vi "P-733 XY Stage Engine.vi"(0 "Notifier Name":string, 11 "Axis Names":string[](array[string])) -> ()   [LabVIEW 2016]
uses:
  Stages Controls/Stage Notifier Element.ctl
  Stages Controls/Stage Actions.ctl
  Stages Controls/Stage Status.ctl
  PI GCS2 DLL/PI_GCS2_DLL_x64.dll
panel:
  in  "Velocity":dbl=5.0
  out "current v":dbl[](array[numeric])
  out "target pos":dbl[](array[numeric])
  out "Success":u32
  in  "Right":bool
  in  "Left":bool
  in  "Y Position (µm)":dbl format="%#.3g"
  in  "Down":bool
  in  "Up":bool
  in  "X Position (µm)":dbl format="%#.3g"
  in  "Step Size (µm)":dbl=0.1
  in  "QUIT":bool
  in  "Abort":bool
  out "P-733 Found":bool
  out "Number Connected":i32
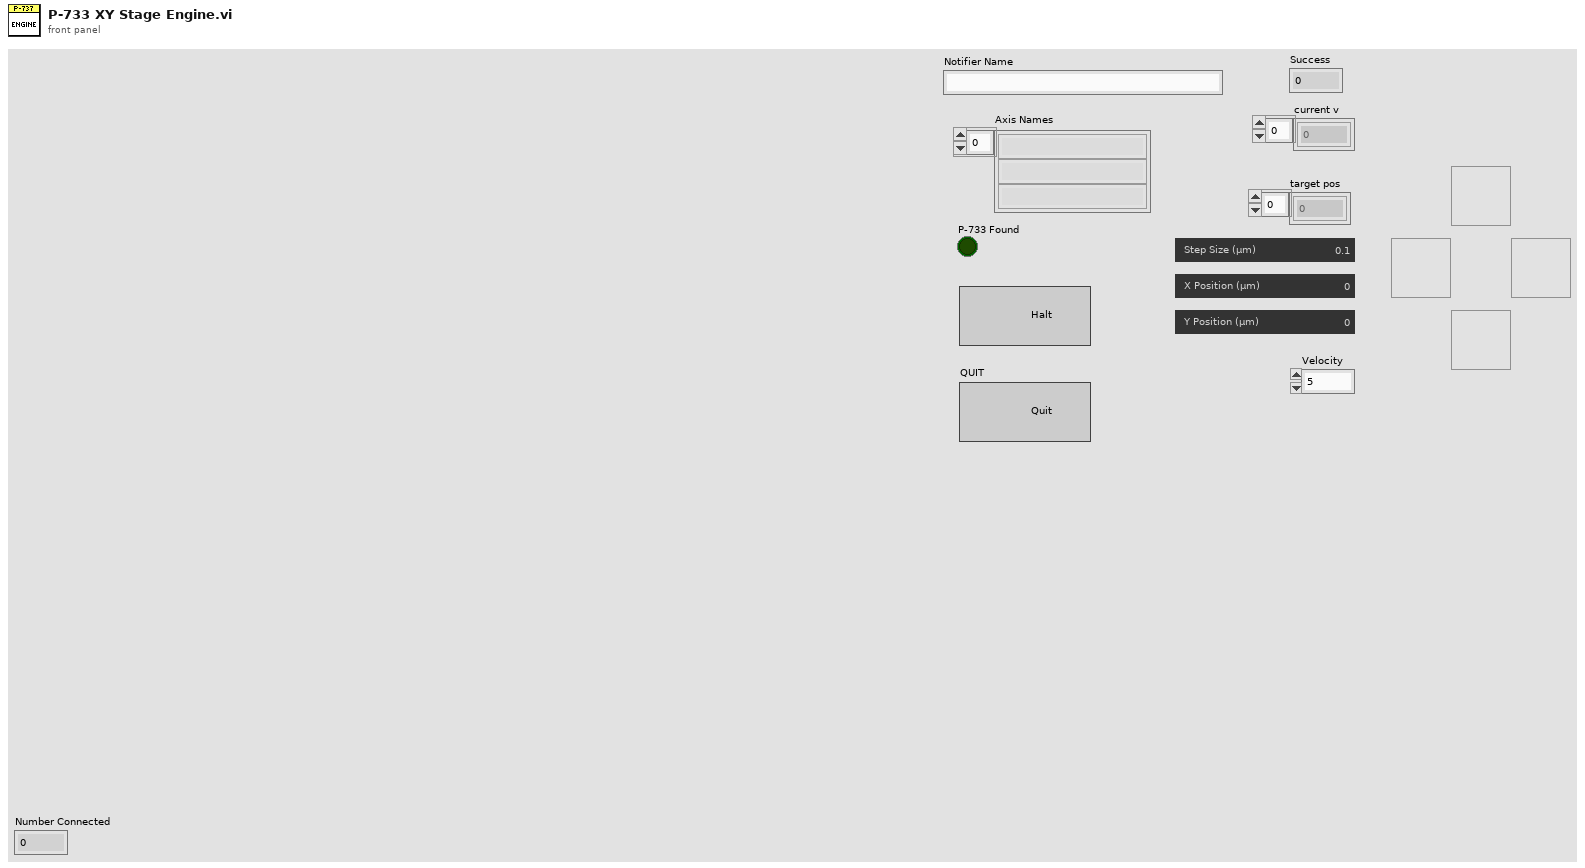
[diagram p1: front panel]
types:
  T1 = typedef "Stage Notifier Element.ctl" = cluster{"Action":T2, "Axis":bool[], "Setpoint":dbl[], "Velocity":dbl, "Cmd Recvd?":bool, "Position":dbl[], "Status":T3, "Misc":variant}
  T2 = typedef "Stage Actions.ctl" = enum16{"Get Position", "MVR", "MOVE", "HALT", "ONTARGET", "ERROR", "REFERENCE", "INIT", "VELOCITY", "STATUS", "EXIT", "HOME", "ZEROPOS", "NANOPOS", "ANALOG", "QUIT"}
  T3 = typedef "Stage Status.ctl" = enum16{"Error", "Abort", "Busy", "On Target"}
  T4 = enum32{"Invalid", "Standard", "Closed", "Hidden", "Minimized", "Maximized"}
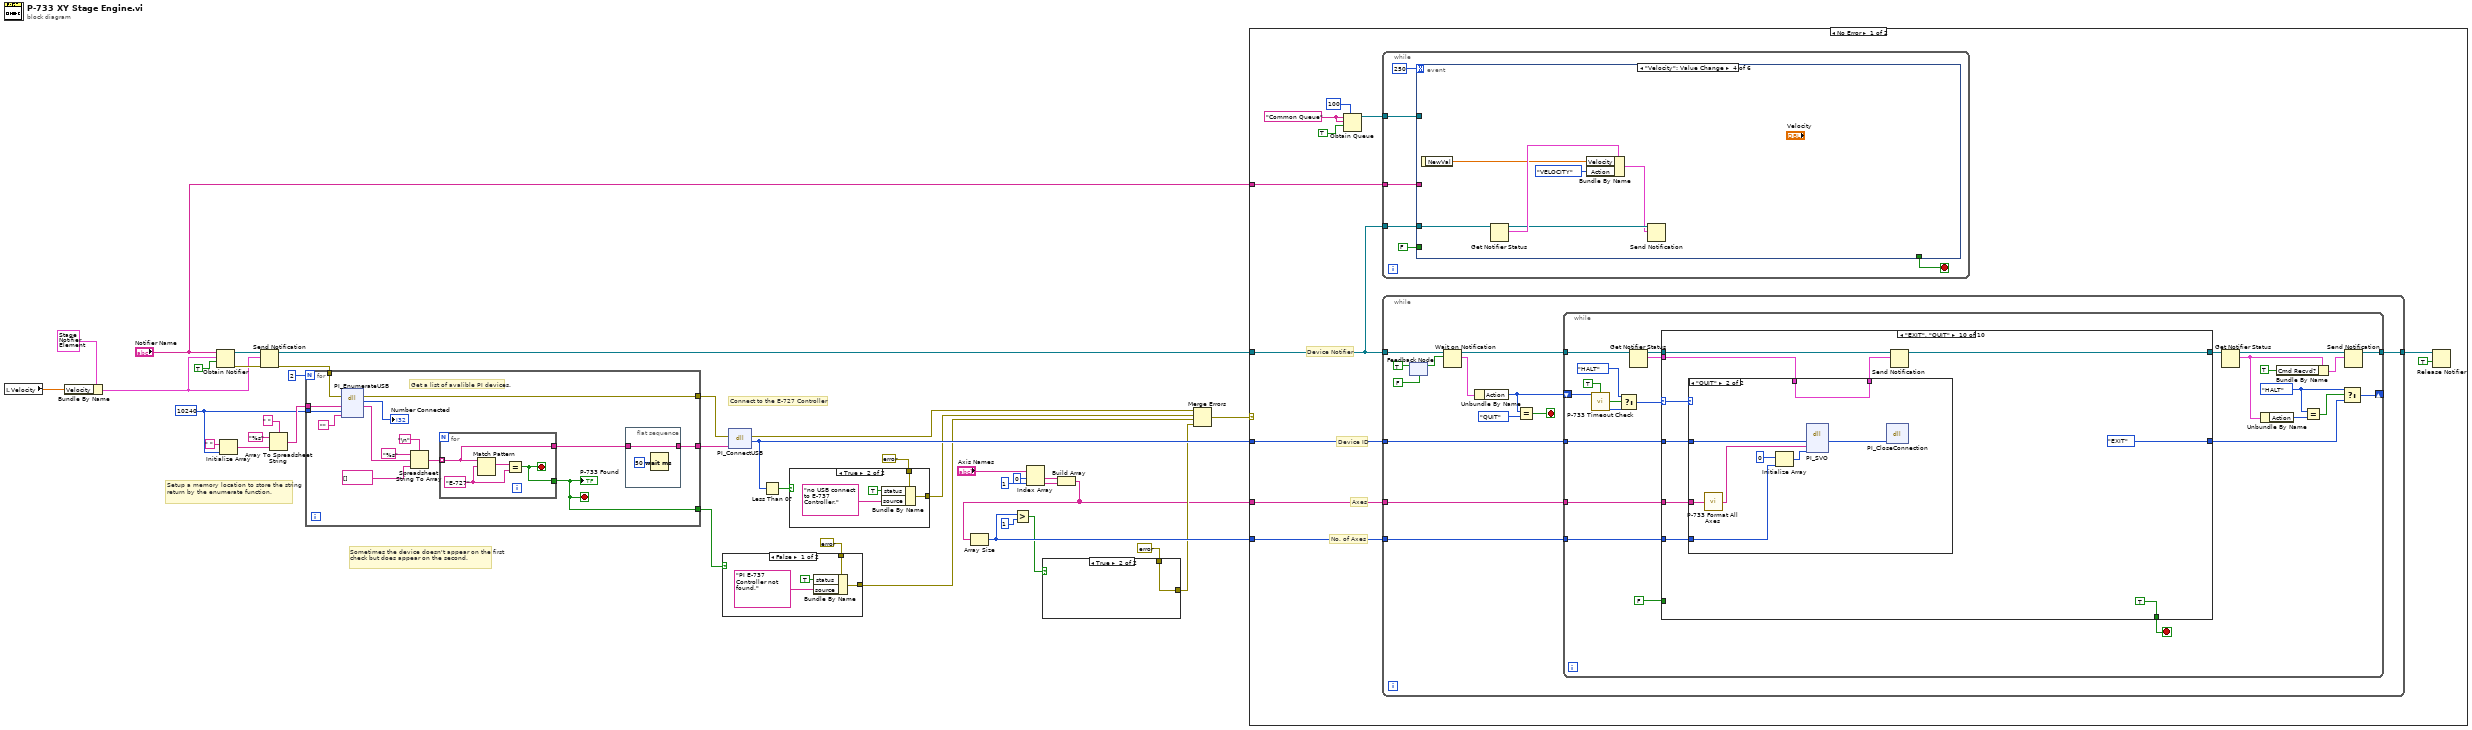
[diagram p0: block diagram]
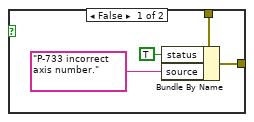
[diagram p2: hidden frame]
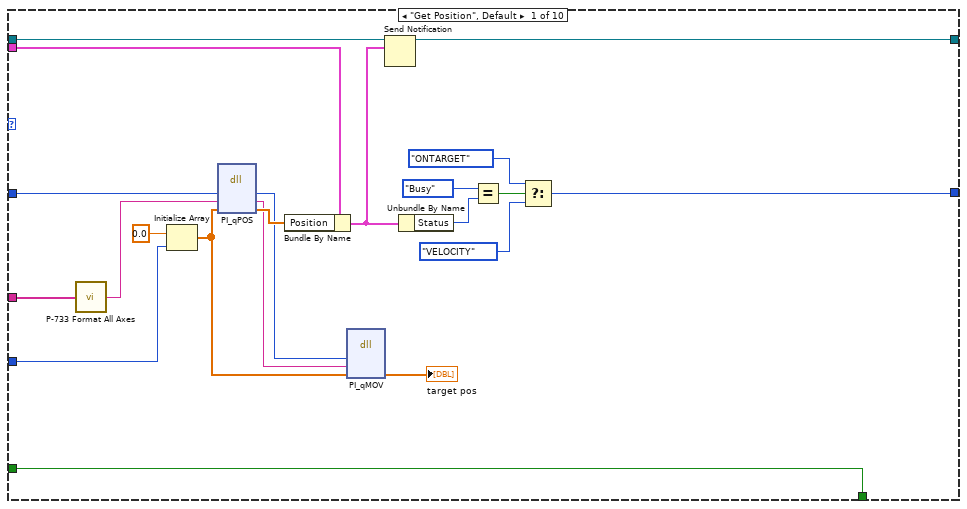
[diagram p5: hidden frame]
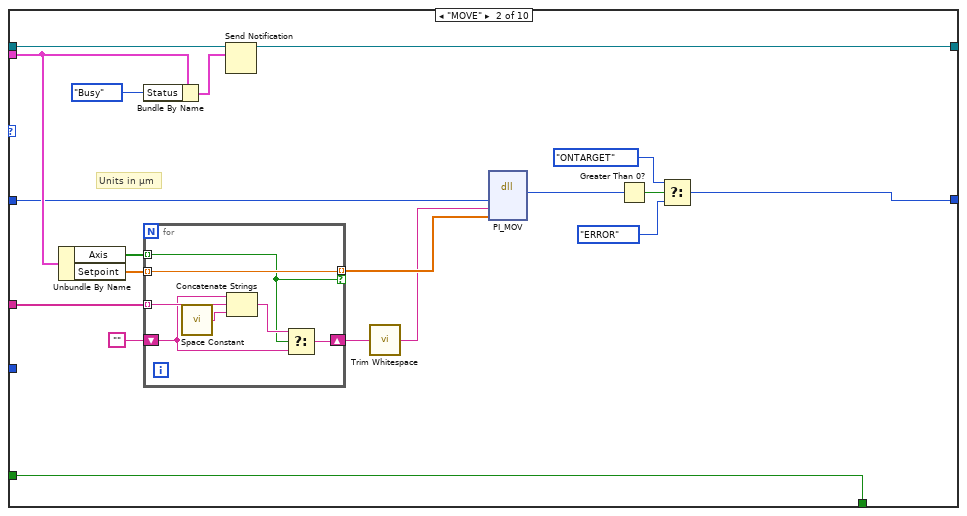
[diagram p6: hidden frame]
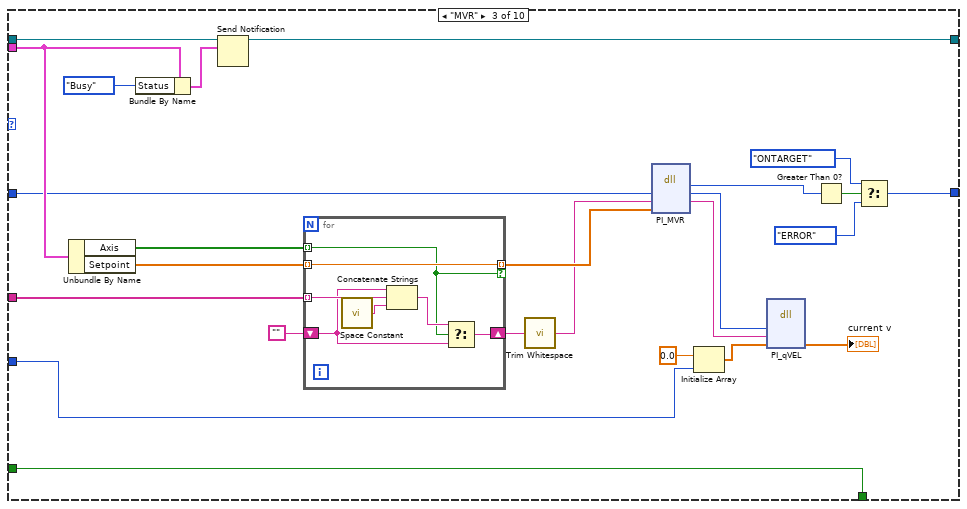
[diagram p7: hidden frame]
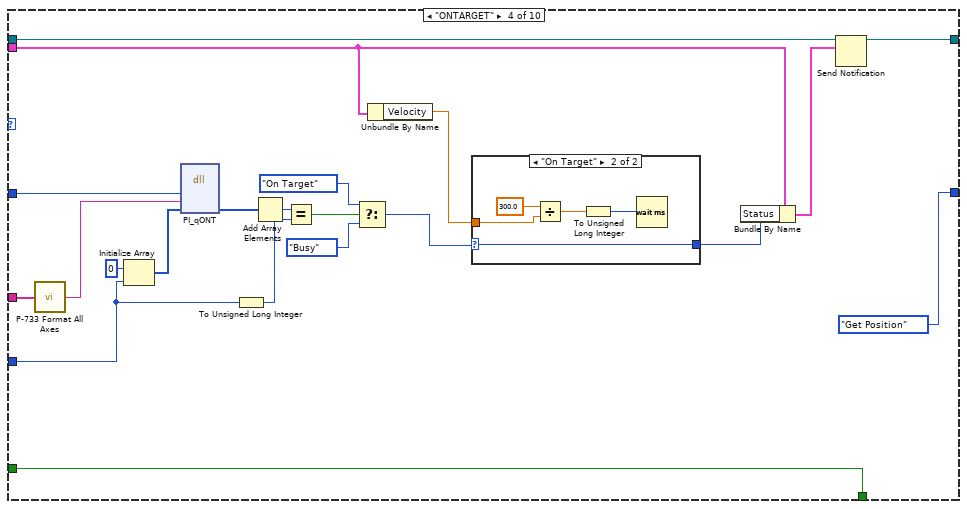
[diagram p8: hidden frame]
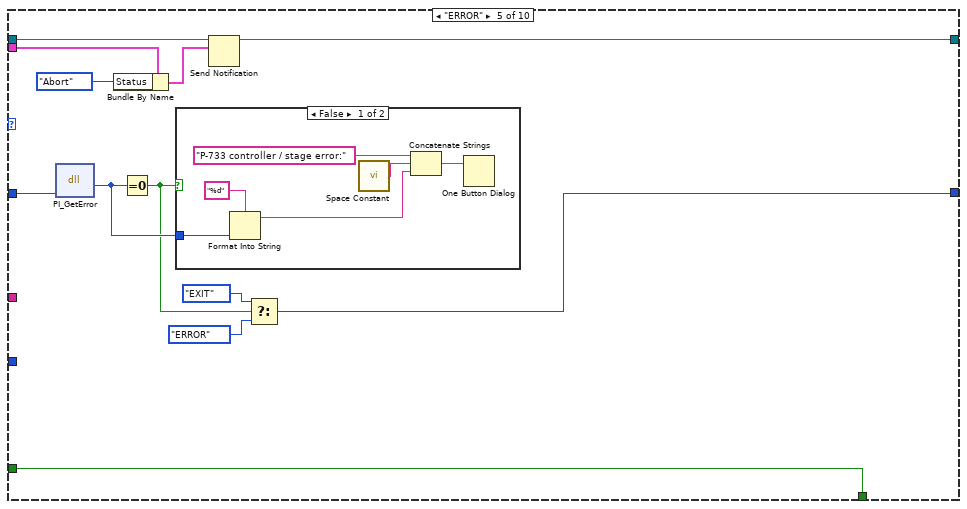
[diagram p10: hidden frame]
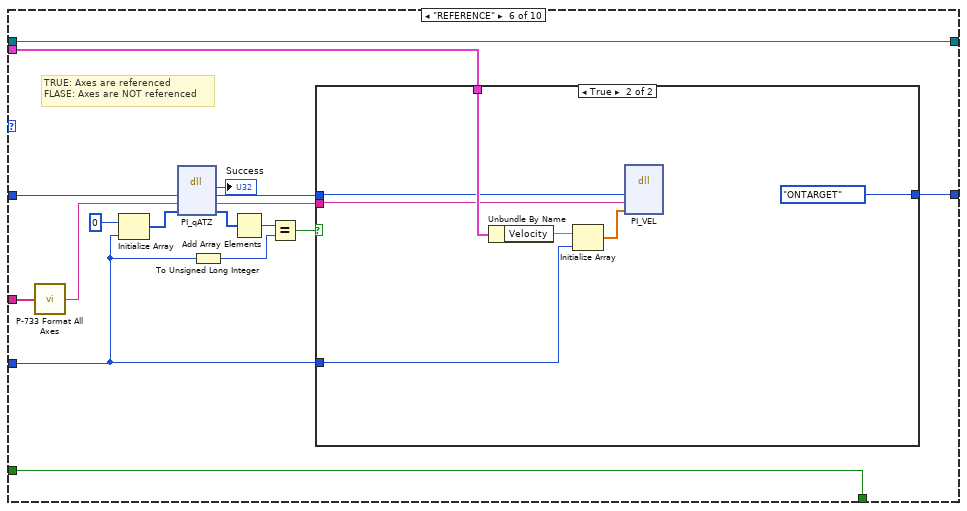
[diagram p12: hidden frame]
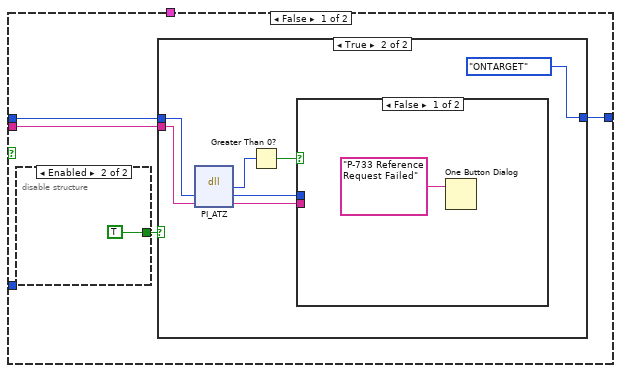
[diagram p13: hidden frame]
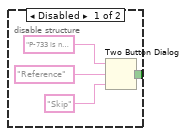
[diagram p14: hidden frame]
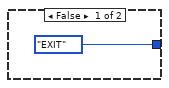
[diagram p15: hidden frame]
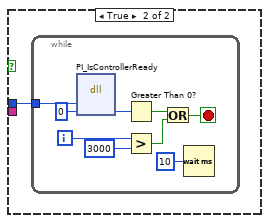
[diagram p16: hidden frame]
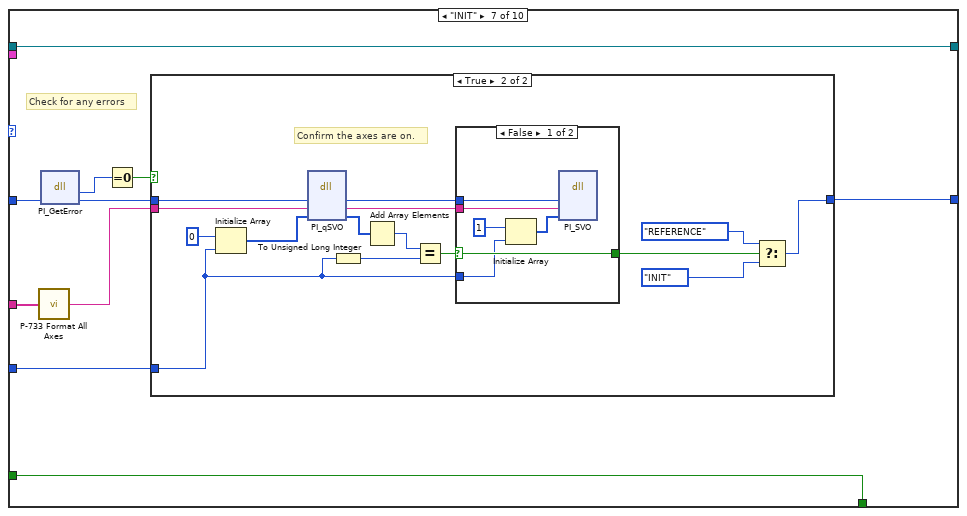
[diagram p17: hidden frame]
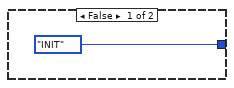
[diagram p18: hidden frame]
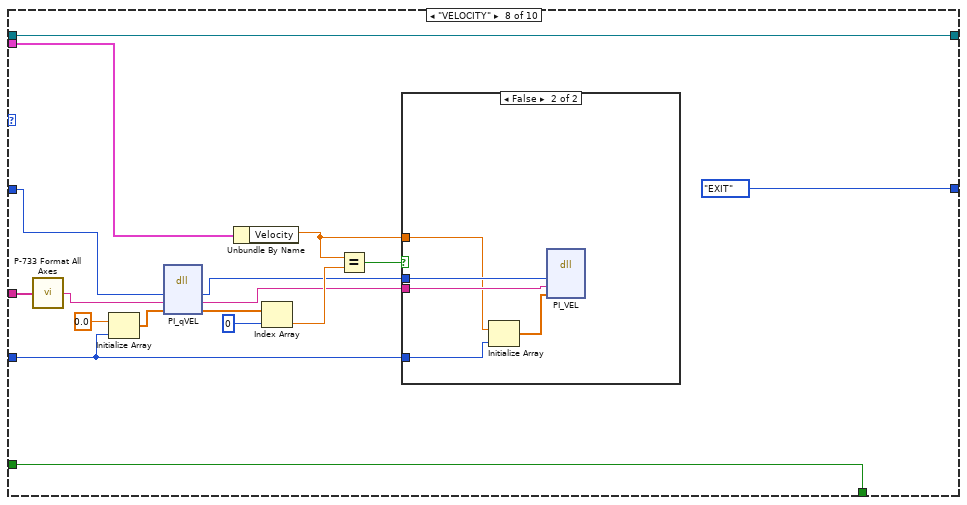
[diagram p20: hidden frame]
diagram:
  w33 = 10240 ("dimension size")
  # "Setup a memory location to store the string return by the enumerate function."
  # "Connect to the E-727 Controller"
  # "Sometimes the device doesn't appear on the first check but does appear on the second."
  n1 = local read "Velocity"() -> (w1:dbl)
  n2 = Bundle By Name(cluster=T1 {"Action"=enum."INIT", "Axis"=[], "Setpoint"=[], "Velocity"=5.0, "Cmd Recvd?"=FALSE, "Position"=[], "Status"=enum."Error", "Misc"=variant} ("Stage Status"), "Velocity"=w1) -> (w2:T1)
  n3 = Obtain Notifier(name (unnamed)="Notifier Name", notification data type=w2, create if not found? (T)=TRUE) -> (notifier out=w19:refnum<notifier>, error out=w18:errorcluster)  [unwired: 1 in, 1 out]
  n4 = Initialize Array(" ", w33) -> (w37:string[])
  n5 = Send Notification(notification=w2, notifier=w19, error in (no error)=w18) -> (notifier out=w16:refnum<notifier>, error out=w17:errorcluster)
  n6 = Array To Spreadsheet String(delimiter (Tab)=" ", array=w37, 3:"%s" ("format string")) -> (spreadsheet string=w34:string)
  n7 = for {
    N: 2 -> [_]
    tunnel: w34 -> [w47]
    tunnel: w33 -> [w46]
    tunnel: [w42] -> w31
    tunnel: [w41] -> w25
    tunnel: [w40] -> w30
    tunnel: w17 -> [w39]
    stop <- w41 stop-if-true
    # "Get a list of avalible PI devices."
    n8 = dll-call lib="C:/Users/Ries Lab/Documents/Microscope Control from Sheng Account/Microscope-Control/Device Library/Stages/PI/PI GCS2 DLL/PI_GCS2_DLL_x64.dll" fn="PI_EnumerateUSB"(error in=w39, "szBuffer"=w47, "iBufferSize"=w46, "szFilter"="") -> (error out=w40:errorcluster, "return type"=→"Number Connected":i32, "szBuffer"=w44:string)  [unwired: 4 in, 1 out]
    n9 = Spreadsheet String To Array(delimiter (Tab)="\n", format string="%s", spreadsheet string=w44, array type (2D Dbl)=string[] []) -> (array=w49:string[])
    n10 = for {
      tunnel: w49 -> [w56] mode=indexing
      tunnel: [w56] -> w43
      tunnel: [w55] -> w41
      stop <- w55 stop-if-true
      w57 = "E-727"
      n11 = Match Pattern(string=w56, regular expression=w57) -> (match substring=w58:string)  [unwired: 1 in, 3 out]
      n12 = Equal?(x=w58, y=w57) -> (x = y?=w55:bool)
    }
    "P-733 Found" <- w41
    n13 = flat-sequence {
      tunnel: w43 -> [w54]
      tunnel: [w54] -> w42
      frame #0 {
        n14 = Wait (ms)(milliseconds to wait=u32 50) -> ()  [unwired: 1 out]
      }
    }
  }
  n15 = case shown="False" w25 {
    tunnel: errorcluster {"status"=FALSE, "code"=0, "source"=""} ("error in (no error)") -> [w60 w63]
    tunnel: [w59 w63] -> w21
    frame False {
      n16 = Bundle By Name(cluster=w60, "status"=TRUE, "source"="PI E-737 Controller not found.") -> (w59:errorcluster)
    }
    frame True {
    }
  }
  n17 = dll-call lib="C:/Users/Ries Lab/Documents/Microscope Control from Sheng Account/Microscope-Control/Device Library/Stages/PI/PI GCS2 DLL/PI_GCS2_DLL_x64.dll" fn="PI_ConnectUSB"(error in=w30, "szDescription"=w31) -> (error out=w23:errorcluster, "Device ID"=w28:i32)  [unwired: 3 in, 1 out]
  n18 = Less Than 0?(x=w28) -> (x < 0?=w27:bool)
  n19 = case shown="True" w27 {
    tunnel: errorcluster {"status"=FALSE, "code"=0, "source"=""} ("error in (no error)") -> [w64 w68]
    tunnel: [w64 w65] -> w22
    frame False {
    }
    frame True {
      n20 = Bundle By Name(cluster=w68, "status"=TRUE, "source"="no USB connect to E-737 Controller.") -> (w65:errorcluster)
    }
  }
  n21 = Index Array(array="Axis Names", index #1=0 ("index"), index #2=1 ("index")) -> (element #1=w6:string, element #2=w5:string)
  n22 = Build Array(w6, w5) -> (w4:string[])
  n23 = Array Size(array=w4) -> (size(s)=w13:i32)
  n24 = Greater?(x=w13, y=1) -> (0:w11:bool)
  n25 = case shown="True" w11 {
    tunnel: errorcluster {"status"=FALSE, "code"=0, "source"=""} ("error in (no error)") -> [w70 w73]
    tunnel: [w69 w73] -> w10
    frame False {
      n26 = Bundle By Name(cluster=w70, "status"=TRUE, "source"="P-733 incorrect axis number.") -> (w69:errorcluster)
    }
    frame True {
    }
  }
  n27 = Merge Errors(w23, w22, w21, w10) -> (w20:errorcluster)
  n28 = case shown="No Error" w20 {
    selector: w20 -> [_ w484]
    tunnel: w16 -> [w78 w486]
    tunnel: "Notifier Name" -> [w79 _]
    tunnel: w28 -> [w77 w485]
    tunnel: w4 -> [w75 _]
    tunnel: w13 -> [w74 _]
    frame No Error {
      w83 = "Common Queue" ("Unique Notifier Name")
      # "Device Notifier"
      # "No. of Axes"
      # "Axes"
      # "Device ID"
      n29 = Obtain Queue(max queue size (-1, unlimited)=100, name (unnamed)=w83, element data type=w83, create if not found? (T)=TRUE) -> (queue out=w80:refnum<queue>)  [unwired: 1 in, 2 out]
      n30 = while {
        tunnel: w78 -> [w386]
        tunnel: w80 -> [w385]
        tunnel: w79 -> [w384]
        stop <- w387 stop-if-true
        n31 = event shown="[3] \"Velocity\": Value Change" {
          selector: _ -> [_ _ _ _ _ _]
          dyn-events: _ -> [_ _ _ _ _ _]
          timeout: 250 -> [_ _ _ _ _ _]
          tunnel: [w398 w407 w425 _ w453 w476] -> w387
          tunnel: w386 -> [w404 _ w418 w439 w445 w479]
          tunnel: w385 -> [w400 _ _ _ _ _]
          tunnel: w384 -> [w395 _ _ _ _ _]
          tunnel: FALSE -> [_ w407 w425 _ w453 w476]
          event Timeout {
            # "Notification with QUIT command"
            n32 = event-data() -> ()  [unwired: 1 in, 1 out]
            n33 = call "Common Device Queue Get Command.vi"("Common Queue"=w400, "Notifier Name"=w395) -> ("Command"=w401:string)  [unwired: 12 in, 1 out]
            n34 = control-ref of="This VI"() -> (w402:refnum<vi>)
            n35 = Get Notifier Status(notifier=w404) -> (notifier out=w396:refnum<notifier>, current notification=w394:T1, error out=w403:errorcluster)  [unwired: 1 in, 2 out]
            n36 = call "Common Device Queue Execute Command.vi"("Common Command"=w401, "VI Refnum"=w402) -> ("Quit?"=w397:bool)  [unwired: 12 in, 1 out]
            n37 = Unbundle By Name(w403) -> ("status"=w399:bool)
            n38 = case shown="True" w397 {
              tunnel: w396 -> [_ w406]
              frame False {
              }
              frame True {
                n39 = Send Notification(notification=T1 {"Action"=enum."QUIT", "Axis"=[], "Setpoint"=[], "Velocity"=5.0, "Cmd Recvd?"=FALSE, "Position"=[], "Status"=enum."Error", "Misc"=variant} ("Stage Status"), notifier=w406) -> ()  [unwired: 1 in, 2 out]
              }
            }
            n40 = Or(x=w397, y=w399) -> (x .or. y?=w398:bool)
            n41 = Unbundle By Name(w394) -> ("Position"=w393:dbl[])
            n42 = Index Array(array=w393, index #1=0 ("index"), index #2=1 ("index")) -> (element #1=w389:dbl, element #2=w390:dbl)
            n43 = local write "X Position (µm)"(w389) -> ()
            n44 = local write "Y Position (µm)"(w390) -> ()
          }
          event Application Instance Close? {
            n45 = event-data() -> ()  [unwired: 1 in, 5 out]
            n46 = control-ref of="This VI"() -> (w409:refnum<vi>)
            n47 = invoke class="VI" method="FP.Open"(reference=w409, "Activate"=TRUE ("Activate?"), "State"=T4."Standard") -> ()  [unwired: 2 in, 5 out]
            n48 = event-data("Discard?"=TRUE) -> ()  [unwired: 1 in, 1 out]
          }
          event "X Position (µm)", "Y Position (µm)": Value Change {
            n49 = event-data() -> ("CtlRef"=w424:refnum<vi>, "NewVal"=w422:dbl)  [unwired: 1 in]
            n50 = Build Array(w422, 0.0) -> (w420:dbl[])
            n51 = property class="DigNum (strict)"(reference=w424) -> ("Label.Text"=w423:string)  [unwired: 1 in, 2 out]
            n52 = case shown="\"Y Position (µm)\"" w423 {
              tunnel: w420 -> [_ w429 w433]
              tunnel: bool[] [TRUE, FALSE] -> [_ w428 w431]
              tunnel: [dbl[] [0.0, 0.0] w429 w432] -> w414
              tunnel: [bool[] [FALSE, FALSE] w428 w430] -> w413
              frame Default {
              }
              frame "X Position (µm)" {
              }
              frame "Y Position (µm)" {
                n53 = Reverse 1D Array(array=w433) -> (reversed array=w432:dbl[])
                n54 = Reverse 1D Array(array=w431) -> (reversed array=w430:bool[])
              }
            }
            n55 = Get Notifier Status(notifier=w418) -> (notifier out=w417:refnum<notifier>, current notification=w416:T1)  [unwired: 1 in, 3 out]
            n56 = Bundle By Name(cluster=w416, "Action"=Stage_Actions."MOVE", "Setpoint"=w414, "Axis"=w413) -> (w412:T1)
            n57 = Send Notification(notification=w412, notifier=w417) -> ()  [unwired: 1 in, 2 out]
          }
          event "Velocity": Value Change {
            n58 = event-data() -> ("NewVal"=w437:dbl)  [unwired: 1 in]
            n59 = Get Notifier Status(notifier=w439) -> (notifier out=w436:refnum<notifier>, current notification=w438:T1)  [unwired: 1 in, 3 out]
            n60 = Bundle By Name(cluster=w438, "Velocity"=w437, "Action"=Stage_Actions."VELOCITY") -> (w435:T1)
            n61 = Send Notification(notification=w435, notifier=w436) -> ()  [unwired: 1 in, 2 out]
          }
          event "Up", "Down", "Left", "Right": Value Change {
            n62 = event-data() -> ("CtlRef"=w448:refnum<vi>)  [unwired: 1 in]
            n63 = property class="Bool"(reference=w448) -> ("Label.Text"=w447:string)  [unwired: 1 in, 2 out]
            n64 = Build Array("Step Size (µm)", 0.0 ("element")) -> (w450:dbl[])
            n65 = case shown="\"Left\", \"Right\"" w447 {
              selector: w447 -> [_ w462 w468]
              tunnel: w450 -> [_ w459 w467]
              tunnel: bool[] [TRUE, FALSE] -> [_ w456 w465]
              tunnel: [dbl[] [0.0, 0.0] w458 w464] -> w442
              tunnel: [bool[] [FALSE, FALSE] w456 w463] -> w441
              frame Default {
              }
              frame "Down", "Up" {
                n66 = Negate(x=w459) -> (-x=w460:dbl[])
                n67 = Equal?(x=w462, y="Down") -> (x = y?=w457:bool)
                n68 = Select(t=w460, s=w457, f=w459) -> (s? t:f=w458:dbl[])
              }
              frame "Left", "Right" {
                n69 = Reverse 1D Array(array=w465) -> (reversed array=w463:bool[])
                n70 = Negate(x=w467) -> (-x=w470:dbl[])
                n71 = Equal?(x=w468, y="Left") -> (x = y?=w469:bool)
                n72 = Select(t=w470, s=w469, f=w467) -> (s? t:f=w466:dbl[])
                n73 = Reverse 1D Array(array=w466) -> (reversed array=w464:dbl[])
              }
            }
            n74 = Get Notifier Status(notifier=w445) -> (notifier out=w446:refnum<notifier>, current notification=w444:T1)  [unwired: 1 in, 3 out]
            n75 = Bundle By Name(cluster=w444, "Action"=Stage_Actions."MVR" ("Actions"), "Setpoint"=w442, "Axis"=w441) -> (w440:T1)
            n76 = Send Notification(notification=w440, notifier=w446) -> ()  [unwired: 1 in, 2 out]
          }
          event "QUIT", "Abort": Value Change {
            n77 = event-data() -> ("CtlRef"=w478:refnum<vi>)  [unwired: 1 in]
            n78 = property class="Bool"(reference=w478) -> ("Label.Text"=w477:string)  [unwired: 1 in, 2 out]
            n79 = case shown="\"QUIT\"" w477 {
              tunnel: [Stage_Actions."EXIT" ("Action") Stage_Actions."QUIT" ("Action") Stage_Actions."HALT" ("Action")] -> w475
              frame "Default", Default {
              }
              frame "QUIT" {
              }
              frame "Abort" {
              }
            }
            n80 = Get Notifier Status(notifier=w479) -> (notifier out=w473:refnum<notifier>, current notification=w472:T1)  [unwired: 1 in, 3 out]
            n81 = Bundle By Name(cluster=w472, "Action"=w475) -> (w474:T1)
            n82 = Send Notification(notification=w474, notifier=w473) -> ()  [unwired: 1 in, 2 out]
          }
        }
      }
      n83 = while {
        tunnel: w78 -> [w96]
        tunnel: w77 -> [w95]
        tunnel: [w93] -> w76
        tunnel: w75 -> [w91]
        tunnel: w74 -> [w90]
        stop <- w92 stop-if-true
        n84 = feedback #1(FALSE) -> (w86:bool)
        n85 = feedback-in #1(TRUE ("ignore previous (F)")) -> ()
        n86 = Wait on Notification(notifier=w96, ignore previous (F)=w86) -> (notifier out=w85:refnum<notifier>, notification=w94:T1)  [unwired: 2 in, 2 out]
        n87 = Unbundle By Name(w94) -> ("Action"=w89:T2)
        n88 = Equal?(x=w89, y=Stage_Actions."QUIT") -> (x = y?=w92:bool)
        n89 = while {
          tunnel: w95 -> [w120]
          tunnel: w85 -> [w117]
          shift-right: [w119] -> _
          shift-left: w89 -> [w113]
          tunnel: [w99] -> w93
          tunnel: w91 -> [w107]
          tunnel: w90 -> [w108]
          stop <- w121 stop-if-true
          w104 = Stage_Actions."HALT" ("t")
          n90 = call "P-733 Timeout Check.vi"("Action"=w113, "User Input?"=TRUE) -> ("Timeout?"=w112:bool, "Action (Dup)"=w111:T2)  [unwired: 12 in]
          n91 = Select(t=Stage_Actions."HALT" ("y"), s=w112, f=w111) -> (s? t:f=w110:T2)
          n92 = Get Notifier Status(notifier=w117) -> (notifier out=w116:refnum<notifier>, current notification=w115:T1)  [unwired: 1 in, 3 out]
          n93 = case shown="\"EXIT\", \"QUIT\"" w110 {
            selector: w110 -> [_ _ _ _ _ _ _ _ _ w371]
            tunnel: w116 -> [w132 w146 w181 w211 w233 w263 w302 w348 w361 w369]
            tunnel: FALSE -> [w142 w162 w194 w222 w240 w262 w306 w347 w354 _]
            tunnel: [w142 w162 w194 w222 w240 w262 w306 w347 w354 TRUE] -> w121
            tunnel: [w136 w158 w190 Stage_Actions."Get Position" ("y") w234 w258 w303 Stage_Actions."EXIT" ("y") Stage_Actions."ERROR" ("y") Stage_Actions."EXIT" ("y")] -> w118
            tunnel: w120 -> [w130 w155 w178 w207 w239 w261 w308 w337 w363 w372]
            tunnel: [w131 w144 w179 w210 w232 w263 w302 w348 w359 w367] -> w106
            tunnel: w115 -> [w135 w156 w188 w203 w231 w248 _ w346 w362 w370]
            tunnel: w108 -> [w124 _ w173 w218 _ w247 w299 w332 _ w364]
            tunnel: w107 -> [w133 w151 w185 w212 _ w251 w301 w344 w357 w365]
            frame "Get Position", Default {
              n94 = call "P-733 Format All Axes.vi"("All Axis Array"=w133) -> ("All Axes String"=w129:string)  [unwired: 14 in]
              n95 = Initialize Array(0.0 ("element"), w124) -> (w126:dbl[])
              n96 = dll-call lib="C:/Users/Ries Lab/Documents/Microscope Control from Sheng Account/Microscope-Control/Device Library/Stages/PI/PI GCS2 DLL/PI_GCS2_DLL_x64.dll" fn="PI_qPOS"("Device ID"=w130, "szAxes"=w129, "pdValueArray"=w126) -> ("Device ID"=w128:i32, "szAxes"=w127:string, "pdValueArray"=w134:dbl[])  [unwired: 4 in, 2 out]
              n97 = Bundle By Name(cluster=w135, "Position"=w134) -> (w123:T1)
              n98 = dll-call lib="C:/Users/Ries Lab/Documents/Microscope Control from Sheng Account/Microscope-Control/Device Library/Stages/PI/PI GCS2 DLL/PI_GCS2_DLL_x64.dll" fn="PI_qMOV"("ID"=w128, "szAxis"=w127, "pdValueArray"=w126) -> ("pdValueArray"=→"target pos":dbl[])  [unwired: 6 in, 2 out]
              n99 = Send Notification(notification=w123, notifier=w132) -> (notifier out=w131:refnum<notifier>)  [unwired: 1 in, 1 out]
              n100 = Unbundle By Name(w123) -> ("Status"=w141:T3)
              n101 = Equal?(x=Stage_Status."Busy", y=w141) -> (x = y?=w139:bool)
              n102 = Select(t=Stage_Actions."ONTARGET" ("y"), s=w139, f=Stage_Actions."VELOCITY" ("y")) -> (s? t:f=w136:T2)
            }
            frame "MOVE" {
              # "Units in µm"
              n103 = Unbundle By Name(w156) -> ("Axis"=w153:bool[], "Setpoint"=w152:dbl[])
              n104 = Bundle By Name(cluster=w156, "Status"=Stage_Status."Busy") -> (w145:T1)
              n105 = for {
                tunnel: w153 -> [w165] mode=indexing
                tunnel: w152 -> [w166] mode=indexing
                tunnel: w151 -> [w169] mode=indexing
                shift-right: [w164] -> w148
                shift-left: "" -> [w163]
                tunnel: [w166] -> w149 mode=indexing if=w165
                n106 = call <vilib>:"Space Constant.vi"() -> ("String"=w168:string)
                n107 = Concatenate Strings(w163, w169, w168) -> (w167:string)
                n108 = Select(t=w167, s=w165, f=w163) -> (s? t:f=w164:string)
              }
              n109 = Send Notification(notification=w145, notifier=w146) -> (notifier out=w144:refnum<notifier>)  [unwired: 1 in, 1 out]
              n110 = call <vilib>:"Trim Whitespace.vi"("string"=w148) -> ("trimmed string"=w147:string)  [unwired: 1 in]
              n111 = dll-call lib="C:/Users/Ries Lab/Documents/Microscope Control from Sheng Account/Microscope-Control/Device Library/Stages/PI/PI GCS2 DLL/PI_GCS2_DLL_x64.dll" fn="PI_MOV"("Device ID"=w155, "szAxes"=w147, "pdValueArray"=w149) -> ("Success"=w154:u32)  [unwired: 6 in, 2 out]
              n112 = Greater Than 0?(x=w154) -> (x > 0?=w161:bool)
              n113 = Select(t=Stage_Actions."ONTARGET" ("Action"), s=w161, f=Stage_Actions."ERROR" ("Action")) -> (s? t:f=w158:T2)
            }
            frame "MVR" {
              n114 = Unbundle By Name(w188) -> ("Axis"=w186:bool[], "Setpoint"=w170:dbl[])
              n115 = Bundle By Name(cluster=w188, "Status"=Stage_Status."Busy") -> (w180:T1)
              n116 = Send Notification(notification=w180, notifier=w181) -> (notifier out=w179:refnum<notifier>)  [unwired: 1 in, 1 out]
              n117 = for {
                tunnel: w186 -> [w197] mode=indexing
                tunnel: w170 -> [w198] mode=indexing
                tunnel: w185 -> [w201] mode=indexing
                shift-right: [w196] -> w182
                shift-left: "" -> [w195]
                tunnel: [w198] -> w183 mode=indexing if=w197
                n118 = call <vilib>:"Space Constant.vi"() -> ("String"=w200:string)
                n119 = Concatenate Strings(w195, w201, w200) -> (w199:string)
                n120 = Select(t=w199, s=w197, f=w195) -> (s? t:f=w196:string)
              }
              n121 = call <vilib>:"Trim Whitespace.vi"("string"=w182) -> ("trimmed string"=w177:string)  [unwired: 1 in]
              n122 = dll-call lib="C:/Users/Ries Lab/Documents/Microscope Control from Sheng Account/Microscope-Control/Device Library/Stages/PI/PI GCS2 DLL/PI_GCS2_DLL_x64.dll" fn="PI_MVR"("Device ID"=w178, "szAxes"=w177, "pdValueArray"=w183) -> ("Success"=w187:u32, "Device ID"=w176:i32, "szAxes"=w175:string)  [unwired: 4 in, 2 out]
              n123 = Initialize Array(0.0 ("element"), w173) -> (w172:dbl[])
              n124 = dll-call lib="C:/Users/Ries Lab/Documents/Microscope Control from Sheng Account/Microscope-Control/Device Library/Stages/PI/PI GCS2 DLL/PI_GCS2_DLL_x64.dll" fn="PI_qVEL"("Device ID"=w176, "szAxes"=w175, "pdValueArray"=w172) -> ("pdValueArray"=→"current v":dbl[])  [unwired: 6 in, 2 out]
              n125 = Greater Than 0?(x=w187) -> (x > 0?=w193:bool)
              n126 = Select(t=Stage_Actions."ONTARGET" ("Action"), s=w193, f=Stage_Actions."ERROR" ("Action")) -> (s? t:f=w190:T2)
            }
            frame "ONTARGET" {
              n127 = call "P-733 Format All Axes.vi"("All Axis Array"=w212) -> ("All Axes String"=w209:string)  [unwired: 14 in]
              n128 = Initialize Array(u32 0 ("element"), w218) -> (w208:u32[])
              n129 = dll-call lib="C:/Users/Ries Lab/Documents/Microscope Control from Sheng Account/Microscope-Control/Device Library/Stages/PI/PI GCS2 DLL/PI_GCS2_DLL_x64.dll" fn="PI_qONT"("Device ID"=w207, "szAxes"=w209, "pdValueArray"=w208) -> ("pdValueArray"=w220:u32[])  [unwired: 6 in, 2 out]
              n130 = To Unsigned Long Integer(number=w218) -> (unsigned 32bit integer=w217:u32)
              n131 = Add Array Elements(numeric array=w220) -> (sum=w219:u32)
              n132 = Equal?(x=w219, y=w217) -> (x = y?=w216:bool)
              n133 = Select(t=Stage_Status."On Target" ("Status"), s=w216, f=Stage_Status."Busy" ("Status")) -> (s? t:f=w206:T3)
              n134 = Unbundle By Name(w203) -> ("Velocity"=w202:dbl)
              n135 = case shown="\"On Target\"" w206 {
                selector: w206 -> [w223 w228]
                tunnel: [w223 w228] -> w204
                tunnel: w202 -> [_ w226]
                frame "Busy", Default {
                }
                frame "On Target" {
                  n136 = Divide(x=300.0, y=w226) -> (x/y=w225:dbl)
                  n137 = To Unsigned Long Integer(number=w225) -> (unsigned 32bit integer=w224:u32)
                  n138 = Wait (ms)(milliseconds to wait=w224) -> ()  [unwired: 1 out]
                }
              }
              n139 = Bundle By Name(cluster=w203, "Status"=w204) -> (w205:T1)
              n140 = Send Notification(notification=w205, notifier=w211) -> (notifier out=w210:refnum<notifier>)  [unwired: 1 in, 1 out]
            }
            frame "ERROR" {
              n141 = dll-call lib="C:/Users/Ries Lab/Documents/Microscope Control from Sheng Account/Microscope-Control/Device Library/Stages/PI/PI GCS2 DLL/PI_GCS2_DLL_x64.dll" fn="PI_GetError"("Device ID"=w239) -> ("Error Code"=w238:i32)  [unwired: 4 in, 2 out]
              n142 = Bundle By Name(cluster=w231, "Status"=Stage_Status."Abort") -> (w230:T1)
              n143 = Equal To 0?(x=w238) -> (x = 0?=w237:bool)
              n144 = case shown="False" w237 {
                tunnel: w238 -> [w244 _]
                frame False {
                  n145 = Format Into String(format string="%d", w244) -> (resulting string=w242:string)  [unwired: 2 in, 1 out]
                  n146 = call <vilib>:"Space Constant.vi"() -> ("String"=w245:string)
                  n147 = Concatenate Strings("P-733 controller / stage error:", w245, w242) -> (w241:string)
                  n148 = One Button Dialog(message=w241) -> ()  [unwired: 1 in, 1 out]
                }
                frame True {
                }
              }
              n149 = Send Notification(notification=w230, notifier=w233) -> (notifier out=w232:refnum<notifier>)  [unwired: 1 in, 1 out]
              n150 = Select(t=Stage_Actions."EXIT", s=w237, f=Stage_Actions."ERROR" ("Action")) -> (s? t:f=w234:T2)
            }
            frame "REFERENCE" {
              # "TRUE: Axes are referenced\nFLASE: Axes are NOT referenced"
              n151 = call "P-733 Format All Axes.vi"("All Axis Array"=w251) -> ("All Axes String"=w250:string)  [unwired: 14 in]
              n152 = Initialize Array(u32 0 ("element"), w247) -> (w259:u32[])
              n153 = dll-call lib="C:/Users/Ries Lab/Documents/Microscope Control from Sheng Account/Microscope-Control/Device Library/Stages/PI/PI GCS2 DLL/PI_GCS2_DLL_x64.dll" fn="PI_qATZ"("Device ID"=w261, "szAxes"=w250, "pdValueArray"=w259) -> ("Success"=→"Success":u32, "Device ID"=w256:i32, "szAxes"=w257:string, "pdValueArray"=w255:u32[])  [unwired: 3 in, 2 out]
              n154 = To Unsigned Long Integer(number=w247) -> (unsigned 32bit integer=w253:u32)
              n155 = Add Array Elements(numeric array=w255) -> (sum=w254:u32)
              n156 = Equal?(x=w254, y=w253) -> (x = y?=w252:bool)
              n157 = case shown="True" w252 {
                tunnel: [w264 Stage_Actions."ONTARGET" ("Action")] -> w258
                tunnel: w257 -> [w265 w293]
                tunnel: w256 -> [w266 w294]
                tunnel: w248 -> [_ w295]
                tunnel: w247 -> [_ w292]
                frame False {
                  n158 = disable-structure shown="Enabled" {
                    disable-tunnel: [w269 TRUE ("T button?")] -> w267
                    frame Disabled {
                      n159 = Two Button Dialog(message="P-733 is not referenced.", 1:"Skip" ("F button name (\"Cancel\")"), 2:"Reference" ("T button name (\"OK\")")) -> (T button?=w269:bool)
                    }
                    frame Enabled {
                    }
                  }
                  n160 = case shown="True" w267 {
                    tunnel: w266 -> [_ w274]
                    tunnel: w265 -> [_ w275]
                    tunnel: [Stage_Actions."EXIT" ("Action") Stage_Actions."ONTARGET" ("Action")] -> w264
                    frame False {
                    }
                    frame True {
                      n161 = dll-call lib="C:/Users/Ries Lab/Documents/Microscope Control from Sheng Account/Microscope-Control/Device Library/Stages/PI/PI GCS2 DLL/PI_GCS2_DLL_x64.dll" fn="PI_ATZ"("Device ID"=w274, "szAxes"=w275) -> ("Success"=w276:u32, "Device ID"=w278:i32, "szAxes"=w279:string)  [unwired: 3 in, 2 out]
                      n162 = Greater Than 0?(x=w276) -> (x > 0?=w277:bool)
                      n163 = case shown="False" w277 {
                        tunnel: w278 -> [_ w282]
                        tunnel: w279 -> [_ _]
                        frame False {
                          n164 = One Button Dialog(message="P-733 Reference Request Failed") -> ()  [unwired: 1 in, 1 out]
                        }
                        frame True {
                          n165 = while {
                            tunnel: w282 -> [w291]
                            i -> [w289]
                            stop <- w284 stop-if-true
                            n166 = dll-call lib="C:/Users/Ries Lab/Documents/Microscope Control from Sheng Account/Microscope-Control/Device Library/Stages/PI/PI GCS2 DLL/PI_GCS2_DLL_x64.dll" fn="PI_IsControllerReady"("Device ID"=w291, "piControllerReady"=0) -> ("piControllerReady"=w287:i32)  [unwired: 5 in, 2 out]
                            n167 = Greater Than 0?(x=w287) -> (x > 0?=w286:bool)
                            n168 = Greater?(x=w289, y=3000) -> (0:w285:bool)
                            n169 = Or(x=w286, y=w285) -> (x .or. y?=w284:bool)
                            n170 = Wait (ms)(milliseconds to wait=u32 10) -> ()  [unwired: 1 out]
                          }
                        }
                      }
                    }
                  }
                }
                frame True {
                  n171 = Unbundle By Name(w295) -> ("Velocity"=w297:dbl)
                  n172 = Initialize Array(w297, w292) -> (w296:dbl[])
                  n173 = dll-call lib="C:/Users/Ries Lab/Documents/Microscope Control from Sheng Account/Microscope-Control/Device Library/Stages/PI/PI GCS2 DLL/PI_GCS2_DLL_x64.dll" fn="PI_VEL"("Device ID"=w294, "szAxes"=w293, "pdValueArray"=w296) -> ()  [unwired: 7 in, 2 out]
                }
              }
            }
            frame "INIT" {
              # "Check for any errors"
              n174 = call "P-733 Format All Axes.vi"("All Axis Array"=w301) -> ("All Axes String"=w300:string)  [unwired: 14 in]
              n175 = dll-call lib="C:/Users/Ries Lab/Documents/Microscope Control from Sheng Account/Microscope-Control/Device Library/Stages/PI/PI GCS2 DLL/PI_GCS2_DLL_x64.dll" fn="PI_GetError"("Device ID"=w308) -> ("Error Code"=w307:i32, "Device ID"=w304:i32)  [unwired: 3 in, 2 out]
              n176 = Equal To 0?(x=w307) -> (x = 0?=w305:bool)
              n177 = case shown="True" w305 {
                tunnel: w304 -> [_ w324]
                tunnel: w300 -> [_ w323]
                tunnel: [Stage_Actions."INIT" ("Action") w321] -> w303
                tunnel: w299 -> [_ w316]
                frame False {
                }
                frame True {
                  # "Confirm the axes are on."
                  n178 = Initialize Array(u32 0 ("element"), w316) -> (w318:u32[])
                  n179 = dll-call lib="C:/Users/Ries Lab/Documents/Microscope Control from Sheng Account/Microscope-Control/Device Library/Stages/PI/PI GCS2 DLL/PI_GCS2_DLL_x64.dll" fn="PI_qSVO"("Device ID"=w324, "szAxes"=w323, "pdValueArray"=w318) -> ("Device ID"=w314:i32, "szAxes"=w315:string, "pdValueArray"=w313:u32[])  [unwired: 4 in, 2 out]
                  n180 = To Unsigned Long Integer(number=w316) -> (unsigned 32bit integer=w310:u32)
                  n181 = Add Array Elements(numeric array=w313) -> (sum=w312:u32)
                  n182 = Equal?(x=w312, y=w310) -> (x = y?=w311:bool)
                  n183 = case shown="False" w311 {
                    selector: w311 -> [w328 w331]
                    tunnel: w315 -> [w329 _]
                    tunnel: w314 -> [w330 _]
                    tunnel: [w328 w331] -> w322
                    tunnel: w316 -> [w326 _]
                    frame False {
                      n184 = Initialize Array(u32 1 ("element"), w326) -> (w325:u32[])
                      n185 = dll-call lib="C:/Users/Ries Lab/Documents/Microscope Control from Sheng Account/Microscope-Control/Device Library/Stages/PI/PI GCS2 DLL/PI_GCS2_DLL_x64.dll" fn="PI_SVO"("Device ID"=w330, "szAxes"=w329, "pdValueArray"=w325) -> ()  [unwired: 7 in, 2 out]
                    }
                    frame True {
                    }
                  }
                  n186 = Select(t=Stage_Actions."REFERENCE" ("Action"), s=w322, f=Stage_Actions."INIT" ("Action")) -> (s? t:f=w321:T2)
                }
              }
            }
            frame "VELOCITY" {
              n187 = call "P-733 Format All Axes.vi"("All Axis Array"=w344) -> ("All Axes String"=w338:string)  [unwired: 14 in]
              n188 = Initialize Array(0.0 ("element"), w332) -> (w340:dbl[])
              n189 = dll-call lib="C:/Users/Ries Lab/Documents/Microscope Control from Sheng Account/Microscope-Control/Device Library/Stages/PI/PI GCS2 DLL/PI_GCS2_DLL_x64.dll" fn="PI_qVEL"("Device ID"=w337, "szAxes"=w338, "pdValueArray"=w340) -> ("Device ID"=w335:i32, "szAxes"=w334:string, "pdValueArray"=w341:dbl[])  [unwired: 4 in, 2 out]
              n190 = Unbundle By Name(w346) -> ("Velocity"=w333:dbl)
              n191 = Index Array(array=w341, index=0) -> (element=w343:dbl)
              n192 = Equal?(x=w333, y=w343) -> (x = y?=w336:bool)
              n193 = case shown="False" w336 {
                tunnel: w335 -> [_ w353]
                tunnel: w334 -> [_ w352]
                tunnel: w333 -> [_ w351]
                tunnel: w332 -> [_ w350]
                frame True {
                }
                frame False {
                  n194 = Initialize Array(w351, w350) -> (w349:dbl[])
                  n195 = dll-call lib="C:/Users/Ries Lab/Documents/Microscope Control from Sheng Account/Microscope-Control/Device Library/Stages/PI/PI GCS2 DLL/PI_GCS2_DLL_x64.dll" fn="PI_VEL"("Device ID"=w353, "szAxes"=w352, "pdValueArray"=w349) -> ()  [unwired: 7 in, 2 out]
                }
              }
            }
            frame "HALT" {
              # "Halt the named axes"
              n196 = call "P-733 Format All Axes.vi"("All Axis Array"=w357) -> ("All Axes String"=w355:string)  [unwired: 14 in]
              n197 = Bundle By Name(cluster=w362, "Status"=Stage_Status."Abort") -> (w360:T1)
              n198 = dll-call lib="C:/Users/Ries Lab/Documents/Microscope Control from Sheng Account/Microscope-Control/Device Library/Stages/PI/PI GCS2 DLL/PI_GCS2_DLL_x64.dll" fn="PI_HLT"("Device ID"=w363, "szAxes"=w355) -> ()  [unwired: 6 in, 2 out]
              n199 = Send Notification(notification=w360, notifier=w361) -> (notifier out=w359:refnum<notifier>)  [unwired: 1 in, 1 out]
            }
            frame "EXIT", "QUIT" {
              n200 = case shown="\"QUIT\"" w371 {
                tunnel: w372 -> [_ w378]
                tunnel: w370 -> [w374 w382]
                tunnel: [w374 w382] -> w368
                tunnel: w365 -> [_ w379]
                tunnel: w364 -> [_ w376]
                frame Default {
                }
                frame "QUIT" {
                  n201 = call "P-733 Format All Axes.vi"("All Axis Array"=w379) -> ("All Axes String"=w377:string)  [unwired: 14 in]
                  n202 = Initialize Array(u32 0 ("element"), w376) -> (w380:u32[])
                  n203 = dll-call lib="C:/Users/Ries Lab/Documents/Microscope Control from Sheng Account/Microscope-Control/Device Library/Stages/PI/PI GCS2 DLL/PI_GCS2_DLL_x64.dll" fn="PI_SVO"("Device ID"=w378, "szAxes"=w377, "pdValueArray"=w380) -> ("Device ID"=w375:i32)  [unwired: 6 in, 2 out]
                  n204 = dll-call lib="C:/Users/Ries Lab/Documents/Microscope Control from Sheng Account/Microscope-Control/Device Library/Stages/PI/PI GCS2 DLL/PI_GCS2_DLL_x64.dll" fn="PI_CloseConnection"("Device ID"=w375) -> ()  [unwired: 5 in, 2 out]
                }
              }
              n205 = Send Notification(notification=w368, notifier=w369) -> (notifier out=w367:refnum<notifier>)  [unwired: 1 in, 1 out]
            }
          }
          n206 = Get Notifier Status(notifier=w106) -> (notifier out=w100:refnum<notifier>, current notification=w98:T1)  [unwired: 1 in, 3 out]
          n207 = Unbundle By Name(w98) -> ("Action"=w105:T2)
          n208 = Bundle By Name(cluster=w98, "Cmd Recvd?"=TRUE) -> (w101:T1)
          n209 = Equal?(x=w104, y=w105) -> (x = y?=w103:bool)
          n210 = Select(t=w104, s=w103, f=w118) -> (s? t:f=w119:T2)
          n211 = Send Notification(notification=w101, notifier=w100) -> (notifier out=w99:refnum<notifier>)  [unwired: 1 in, 1 out]
        }
      }
      n212 = Release Notifier(notifier=w76, force destroy? (F)=TRUE) -> ()  [unwired: 1 in, 3 out]
    }
    frame Error {
      n213 = dll-call lib="C:/Users/Ries Lab/Documents/Microscope Control from Sheng Account/Microscope-Control/Device Library/Stages/PI/PI GCS2 DLL/PI_GCS2_DLL_x64.dll" fn="PI_CloseConnection"(error in=w484, "Device ID"=w485) -> (error out=w483:errorcluster)  [unwired: 4 in, 1 out]
      n214 = Release Notifier(notifier=w486, force destroy? (F)=TRUE, error in (no error)=w483) -> (error out=w491:errorcluster)  [unwired: 2 out]
      n215 = Unbundle By Name(w491) -> ("source"=w488:string)
      n216 = Concatenate Strings("P-733 Initialization Error", "\r", w488) -> (w487:string)
      n217 = One Button Dialog(message=w487) -> ()  [unwired: 1 in, 1 out]
    }
  }
